vi "FIFO_ReadBlock.vi"(8 "error in (no error)":errorcluster, 11 "rt fifo ref in":refnum<k33>) -> (0 "error out":errorcluster, 1 "blok?":bool, 2 "dane":i16[][](array[numeric]), 3 "rt fifo ref out":refnum<k33>)   [LabVIEW 2025]
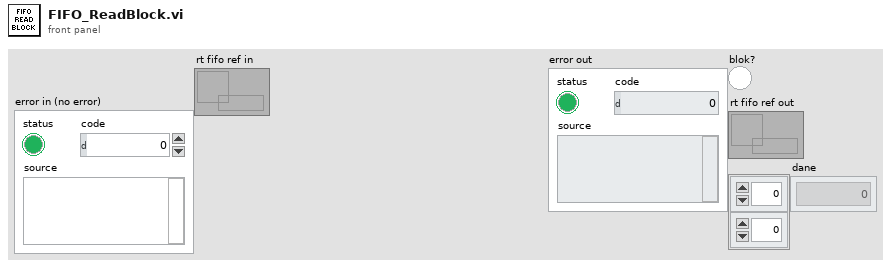
[diagram p1: front panel]
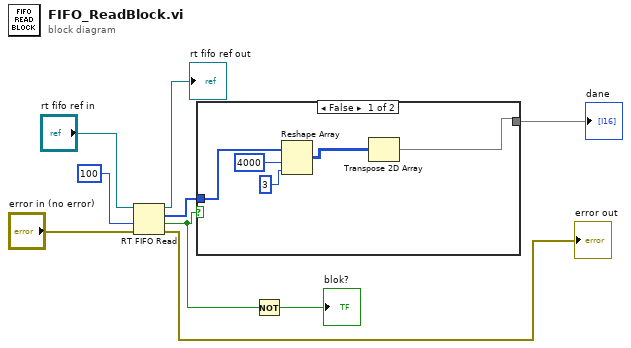
[diagram p0: block diagram]
diagram:
  n1 = RT FIFO Read(0:"rt fifo ref in", 2:100 ("timeout in ms (0)"), 3:"error in (no error)") -> (8:→"rt fifo ref out":refnum<k33>, 9:w7:i16[], 10:w2:bool, 11:→"error out":errorcluster)  [unwired: 1 in, 1 out]
  n2 = case shown="False" w2 {
    tunnel: w7 -> [w14 _]
    tunnel: [w10 _] -> w4
    frame False {
      n3 = Reshape Array(w14, 4000 ("dimension size"), 3 ("dimension size")) -> (w11:i16[][])
      n4 = Transpose 2D Array(2D array=w11) -> (transposed array=w10:i16[][])
    }
    frame True {
    }
  }
  "dane" <- w4
  n5 = Not(x=w2) -> (.not. x?=→"blok?":bool)
